vi "SIL Simulation.vi"(11 "Bus Access":refnum<class "Bus_Access.lvclass">[](array[class])) -> ()   [LabVIEW 2021]
uses:
  <vilib>/TSA/Omni-Bus/Omni-Bus/Bus Access/Bus_Access.lvclass
  <vilib>/TSA/Omni-Bus/Omni-Bus/Omni_Bus.lvclass
  <vilib>/TSA/Omni-Bus/Omni-Bus/Support/Read/Read DBL.vi
  <vilib>/TSA/Omni-Bus/Omni-Bus/Support/Read/Read Boolean.vi
  <vilib>/TSA/Omni-Bus/Omni-Bus/Support/Write/Write DBL.vi
  <vilib>/TSA/Abstract Data Classes/Abs_Types/Double Float/Abs_Double Float.lvclass
  C:/Program Files (x86)/National Instruments/LabVIEW 2021/vi.lib/TSA/Abstract Data Classes/Abs_Types/Type/Abs_Type.lvclass
  <vilib>/TSA/Abstract Data Classes/Abs_Types/Boolean/Abs_Boolean.lvclass
  <vilib>/TSA/Omni-Bus/Omni-Bus/Support/FindVar.vi
  <vilib>/ptbypt/NI_PtbyPt.lvlib
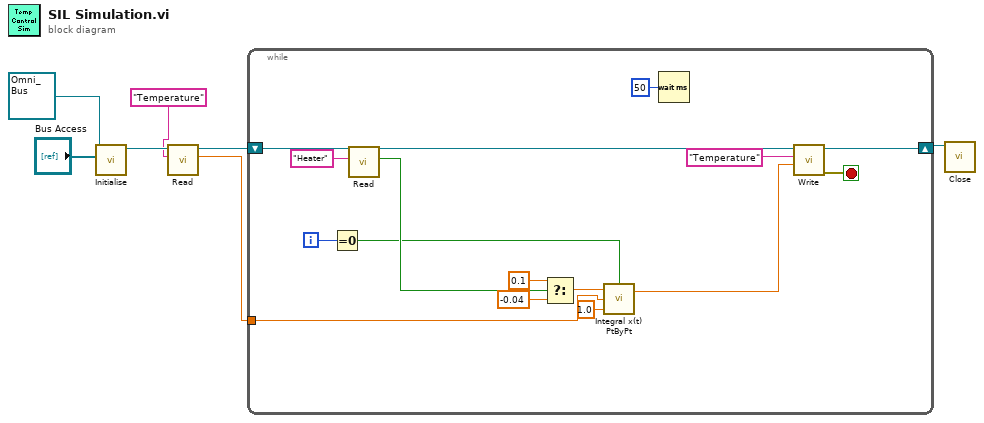
[diagram p0: block diagram]
diagram:
  n1 = call-dynamic "Initialise.vi"("Bus Access"="Bus Access", "Var Bus in"=refnum<class "Omni_Bus.lvclass"> refnum) -> ("Var Bus out"=w4:refnum<class "Omni_Bus.lvclass">)  [unwired: 8 in, 1 out]
  n2 = call-poly <vilib>:"Read.vi"("Tag"="Temperature", "Var Bus in"=w4) -> ("Numeric"=w1:dbl, "Var Bus out"=w3:refnum<class "Omni_Bus.lvclass">)  [unwired: 7 in, 1 out]
  n3 = while {
    shift-right: [w18] -> w6
    shift-left: w3 -> [w20]
    tunnel: w1 -> [w8]
    i -> [w10]
    stop <- w17 stop-if-true
    n4 = Equal To 0?(x=w10) -> (x = 0?=w9:bool)
    n5 = call-poly <vilib>:"Read.vi"("Tag"="Heater", "Var Bus in"=w20) -> ("Boolean"=w16:bool, "Var Bus out"=w19:refnum<class "Omni_Bus.lvclass">)  [unwired: 7 in, 1 out]
    n6 = Select(t=0.1, s=w16, f=-0.04) -> (s? t:f=w14:dbl)
    n7 = call <vilib>:"Integral x(t) PtByPt.vi"("initialize"=w9, "dt"=1.0, "initial condition"=w8, "x"=w14) -> ("integral x(t)"=w15:dbl)  [unwired: 1 out]
    n8 = Wait (ms)(milliseconds to wait=u32 50) -> ()  [unwired: 1 out]
    n9 = call-poly <vilib>:"Write.vi"("Numeric"=w15, "Tag"="Temperature", "Omni_Bus in"=w19) -> ("error out"=w17:errorcluster, "Omni_Bus out"=w18:refnum<class "Omni_Bus.lvclass">)  [unwired: 7 in]
  }
  n10 = call-dynamic "Close.vi"("Data in"=w6) -> ()  [unwired: 9 in, 2 out]
